vi "Read Resource Contents.vi"(8 "error in":errorcluster, 9 "file path":path, 10 "mimeType":string, 11 "uri":string) -> (0 "error out":errorcluster, 3 "result":string)   [LabVIEW 2020, in "MCP Server.lvlib"]
doc: "Builds the result of resources/read for one file resource.\n\nThe file is read byte for byte. For a binary MIME type (application/pdf, image/gif, image/jpeg, image/png) the bytes are returned Base64 encoded in blob. For every other MIME type the bytes are taken as UTF-8 text and returned in text as one JSON string, with the line endings of the file.\n\nresult is {\"contents\":[{\"uri\":...,\"mimeType\":...,\"text\" or \"blob\":...}]}."
uses:
  MCP Server.lvlib
  f3e7ecff-b872-4694-956c-e6c1c4e92882.vi
  20d5451d-7b82-49a2-bb37-1ca74be373ec.vi
  <vilib>/JDP Science/JSONtext/support/Quote and Escape JSON string.vi
  <vilib>/JDP Science/JSONtext/support/quote and escape json string 2.vi
  <vilib>/JDP Science/JSONtext/Variant to JSON Text.vi
  <vilib>/JDP Science/JSONtext/LVClass Serializer/JSONtext LVClass Serializer.lvclass
  <vilib>/JDP Science/JSONtext/JSONtext.lvlib
  <vilib>/JDP Science/JDP Science Common Utilities/Base64/Base64 Support.lvlib
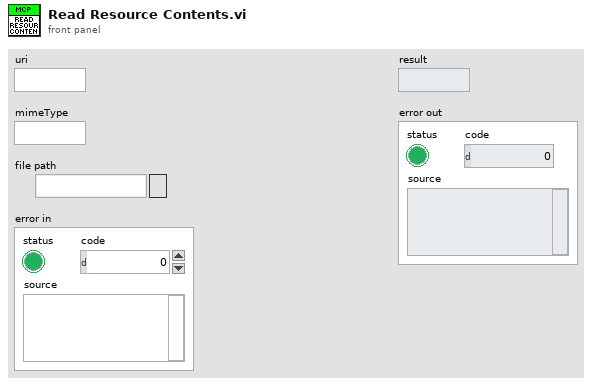
[diagram p1: front panel]
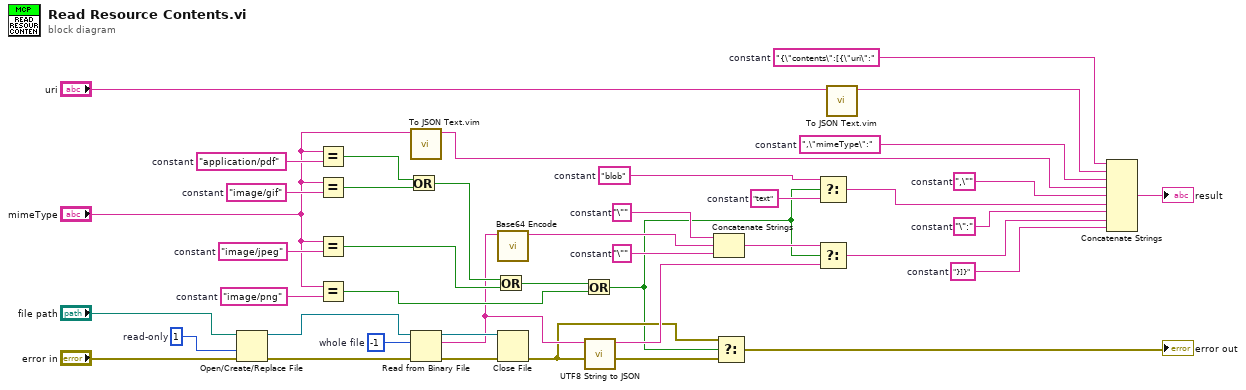
[diagram p0: block diagram]
diagram:
  w6 = "}]}"  # constant
  w8 = "\":"  # constant
  w10 = ",\""  # constant
  w12 = ",\"mimeType\":"  # constant
  w14 = "{\"contents\":[{\"uri\":"  # constant
  w19 = "text"  # constant
  w20 = "blob"  # constant
  w21 = "\""  # constant
  w23 = "\""  # constant
  w31 = "image/png"  # constant
  w32 = "image/jpeg"  # constant
  w33 = "image/gif"  # constant
  w34 = "application/pdf"  # constant
  w38 = -1  # whole file
  w41 = u32 1  # read-only
  n1 = Open/Create/Replace File(file path (use dialog)="file path", error in="error in", access (0:read/write)=w41) -> (refnum out=w39:refnum<file>, error out=w37:errorcluster)  [unwired: 3 in, 1 out]
  n2 = Equal?(x="mimeType", y=w34) -> (x = y?=w30:bool)
  n3 = Equal?(x="mimeType", y=w33) -> (x = y?=w29:bool)
  n4 = Equal?(x="mimeType", y=w32) -> (x = y?=w27:bool)
  n5 = Equal?(x="mimeType", y=w31) -> (x = y?=w25:bool)
  n6 = Or(x=w30, y=w29) -> (x .or. y?=w28:bool)
  n7 = call "To JSON Text.vim"("Anything"="mimeType") -> ("<JSON>"=w11:string)  [unwired: 9 in, 1 out]
  n8 = Read from Binary File(8:w37, 10:w38, 11:w39) -> (0:w35:errorcluster, 2:w24:string, 3:w36:refnum<file>)  [unwired: 3 in, 1 out]
  n9 = Or(x=w28, y=w27) -> (x .or. y?=w26:bool)
  n10 = call <vilib>:"Base64 Encode.vi"("String to Encode"=w24) -> ("Base64 Encoded"=w22:string)  [unwired: 10 in]
  n11 = Close File(refnum=w36, error in=w35) -> (error out=w4:errorcluster)  [unwired: 1 out]
  n12 = Or(x=w26, y=w25) -> (x .or. y?=w3:bool)
  n13 = call <vilib>:"UTF8 String to JSON.vi"("error in (no error)"=w4, "UTF8 String"=w24) -> ("error out"=w2:errorcluster, "<JSON>"=w17:string)  [unwired: 8 in]
  n14 = Concatenate Strings(w23, w22, w21) -> (w18:string)
  n15 = Select(t=w4, s=w3, f=w2) -> (s? t:f=→"error out":errorcluster)
  n16 = Select(t=w20, s=w3, f=w19) -> (s? t:f=w9:string)
  n17 = Select(t=w18, s=w3, f=w17) -> (s? t:f=w7:string)
  n18 = call "To JSON Text.vim"("Anything"="uri") -> ("<JSON>"=w13:string)  [unwired: 9 in, 1 out]
  n19 = Concatenate Strings(w14, w13, w12, w11, w10, w9, w8, w7, w6) -> (→"result":string)
